vi "Sensor_Open.vi"   [LabVIEW 2016]
uses:
  <vilib>/Rock Robotics/SystemInterfaces/AI/FPGA_AIChannel.ctl
  <vilib>/Rock Robotics/SystemInterfaces/DIO/FPGA_DIOChannel.ctl
  <vilib>/Rock Robotics/SystemInterfaces/spilib/spi_bus.ctl
  Sensors/PixyCam/Private/PixyCam_CommMode.ctl
  Sensors/ADI MXP IMU/ADIS16448_IMU.lvlib
  Sensors/PixyCam/PixyCam_LabVIEW.lvlib
  ArgosLib/ArgosLib.lvlib
types:
  T1 = typedef "FPGA_DIOChannel.ctl" = enum8{"DIO 0", "DIO 1", "DIO 2", "DIO 3", "DIO 4", "DIO 5", "DIO 6", "DIO 7", "DIO 8", "DIO 9", "DIO MXP 0", "DIO MXP 1", "DIO MXP 2", "DIO MXP 3", "DIO MXP 4", "DIO MXP 5", "DIO MXP 6", "DIO MXP 7", "DIO MXP 8", "DIO MXP 9", "DIO MXP 10", "DIO MXP 11", "DIO MXP 12", "DIO MXP 13", "DIO MXP 14", "DIO MXP 15", "SPI Port CS1", "SPI Port CS2", "SPI Port CS3", "SPI Port MISO", "SPI Port MOSI", "Invalid"}
  T2 = typedef "spi_bus.ctl" = enum16{"SPI On-Board, CS0", "SPI On-Board, CS1", "SPI On-Board, CS2", "SPI On-Board, CS3", "SPI MXP", "Invalid"}
  T3 = typedef "PixyCam_LabVIEW.lvlib/PixyCam_CommMode.ctl" = enum16{"SPI", "I2C", "UART", "Analog", "Digital"}
  T4 = typedef "FPGA_AIChannel.ctl" = enum8{"AI 0", "AI 1", "AI 2", "AI 3", "AI MXP 0", "AI MXP 1", "AI MXP 2", "AI MXP 3", "Invalid"}
  T5 = typedef "WPI_DigitalInputDevRef.ctl" = cluster{"DevStatus":errorcluster, "DIO Channel":T1}
  T6 = typedef "WPI_AnalogChannelDevRef.ctl" = cluster{"DevStatus":errorcluster, "Analog Channel":T4}
  T7 = typedef "WPI_SonarMB1010DigitalDeviceRef.ctl" = cluster{"CounterDevRef":T8, "Scaling factor (s/in)":dbl}
  T8 = typedef "WPI_CounterDevRef.ctl" = cluster{"DevStatus":errorcluster, "CntIndex":T9}
  T9 = typedef "FPGA_CounterCtrSystemIndex.ctl" = enum8{"Ctr 0", "Ctr 1", "Ctr 2", "Ctr 3", "Ctr 4", "Ctr 5", "Ctr 6", "Ctr 7", "Invalid"}
  T10 = typedef "PixyCam_LabVIEW.lvlib/PixyCam_DevRef.ctl" = cluster{"PixyCamDevRef_SPI":T11, "Communication Mode":T3, "Error":errorcluster}
  T11 = typedef "PixyCam_LabVIEW.lvlib/PixyCam_SPI_DevRef.ctl" = cluster{"SPIDevRef":T12, "Output Queue":refnum<queue>}
  T12 = typedef "WPI_SPIDevRef.ctl" = cluster{"DevStatus":errorcluster, "Handle":i32, "SPI Bus":T2}
  T13 = typedef "ADIS16448_IMU.lvlib/ADI_IMU_ADIS16448_InterruptDevRef.ctl" = cluster{"ADI IMU DevRef":T14, "InterruptRef":T15}
  T14 = typedef "ADIS16448_IMU.lvlib/ADI_IMU_ADIS16448_IMUDevRef.ctl" = cluster{"DevStatus":errorcluster, "Handle":i32, "SPI Bus":T2, "Device Found":bool, "Device Ready":bool, "Yaw Axis":enum16{"X", "Y", "Z"}, "AHRS Algorithm":enum16{"Complementary", "Madgwick"}, "Serial":u16, "Lot ID 2":u16, "Lot ID 1":u16, "Product ID":u16}
  T15 = typedef "WPI_InterruptRef.ctl" = cluster{"DevStatus":errorcluster, "InterruptIndex":T16}
  T16 = typedef "FPGA_InterruptIndex.ctl" = enum8{"0", "1", "2", "3", "4", "5", "6", "7", "Invalid"}
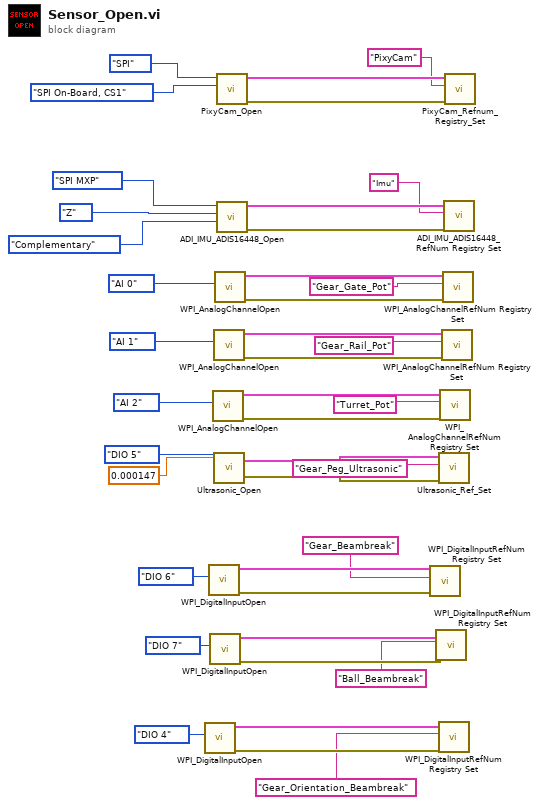
[diagram p0: block diagram]
diagram:
  n1 = call <vilib>:"WPI_DigitalInputOpen.vi"("DIO Channel"=FPGA_DIOChannel."DIO 4") -> ("error out"=w2:errorcluster, "DigitalInputDevRef"=w3:T5)  [unwired: 9 in]
  n2 = call <vilib>:"WPI_DigitalInputOpen.vi"("DIO Channel"=FPGA_DIOChannel."DIO 6") -> ("error out"=w23:errorcluster, "DigitalInputDevRef"=w24:T5)  [unwired: 9 in]
  n3 = call <vilib>:"WPI_DigitalInputOpen.vi"("DIO Channel"=FPGA_DIOChannel."DIO 7") -> ("error out"=w18:errorcluster, "DigitalInputDevRef"=w17:T5)  [unwired: 9 in]
  n4 = call <vilib>:"WPI_AnalogChannelOpen.vi"("Analog Channel"=FPGA_AIChannel."AI 2") -> ("error out"=w33:errorcluster, "AIDeviceRef"=w34:T6)  [unwired: 9 in]
  n5 = call <vilib>:"WPI_AnalogChannelOpen.vi"("Analog Channel"=FPGA_AIChannel."AI 1") -> ("error out"=w32:errorcluster, "AIDeviceRef"=w35:T6)  [unwired: 9 in]
  n6 = call "Ultrasonic_Open.vi"("DIO Channel"=FPGA_DIOChannel."DIO 5", "Scaling factor (s/in)"=0.000147) -> ("error out"=w26:errorcluster, "SonarMB1010DigitalDevRef"=w27:T7)  [unwired: 1 in]
  n7 = call <vilib>:"WPI_AnalogChannelOpen.vi"("Analog Channel"=FPGA_AIChannel."AI 0") -> ("error out"=w31:errorcluster, "AIDeviceRef"=w36:T6)  [unwired: 9 in]
  n8 = call "PixyCam_Open.vi"("SPI Bus"=spi_bus."SPI On-Board, CS1", "Communication Mode"=PixyCam_CommMode."SPI") -> ("error out"=w8:errorcluster, "output cluster"=w7:T10)  [unwired: 4 in]
  n9 = call "ADI_IMU_ADIS16448_Open.vi"("AHRS Algorithm"=enum16{"Complementary", "Madgwick"}."Complementary", "Yaw Axis"=enum16{"X", "Y", "Z"}."Z", "SPI Chip Select"=spi_bus."SPI MXP") -> ("error out"=w12:errorcluster, "ADI IMU Interrupt DevRef"=w13:T13)  [unwired: 7 in]
  n10 = call <vilib>:"WPI_DigitalInputRefNum Registry Set.vi"("error in (no error)"=w23, "refnum name"="Gear_Beambreak", "DigitalInputDevRef"=w24) -> ()  [unwired: 7 in, 2 out]
  n11 = call <vilib>:"WPI_DigitalInputRefNum Registry Set.vi"("error in (no error)"=w18, "refnum name"="Ball_Beambreak", "DigitalInputDevRef"=w17) -> ()  [unwired: 7 in, 2 out]
  n12 = call "Ultrasonic_Ref_Set.vi"("error in (no error)"=w26, "refnum name"="Gear_Peg_Ultrasonic", "SonarMB1010DigitalDevRef 2"=w27) -> ()  [unwired: 1 in, 2 out]
  n13 = call <vilib>:"WPI_DigitalInputRefNum Registry Set.vi"("error in (no error)"=w2, "refnum name"="Gear_Orientation_Beambreak", "DigitalInputDevRef"=w3) -> ()  [unwired: 7 in, 2 out]
  n14 = call <vilib>:"WPI_AnalogChannelRefNum Registry Set.vi"("error in (no error)"=w33, "refnum name"="Turret_Pot", "AIDeviceRef"=w34) -> ()  [unwired: 7 in, 2 out]
  n15 = call <vilib>:"WPI_AnalogChannelRefNum Registry Set.vi"("error in (no error)"=w32, "refnum name"="Gear_Rail_Pot", "AIDeviceRef"=w35) -> ()  [unwired: 7 in, 2 out]
  n16 = call <vilib>:"WPI_AnalogChannelRefNum Registry Set.vi"("error in (no error)"=w31, "refnum name"="Gear_Gate_Pot", "AIDeviceRef"=w36) -> ()  [unwired: 7 in, 2 out]
  n17 = call "ADI_IMU_ADIS16448_RefNum Registry Set.vi"("error in (no error)"=w12, "refnum name"="Imu", "ADI IMU Interrupt DevRef"=w13) -> ()  [unwired: 7 in, 2 out]
  n18 = call "PixyCam_Refnum_Registry_Set.vi"("error in (no error)"=w8, "refnum name"="PixyCam", "PixyCamDevRef"=w7) -> ()  [unwired: 3 in, 2 out]
